vi "Variable glob Leybold.vi"() -> ()   [LabVIEW 2022 SP3]
panel:
  in  "Donnees Leybold":string[](array[string])
  in  "Nom select Leybold":string[](array[string])
  in  "Selection Leybold":bool[](array[boolean])
  in  "Noms Leybold":string[](array[string])
  in  "LEYBOLD":bool
  in  "Port RS232 Leybold":refnum<visa-resource-name>[](array[refnum])
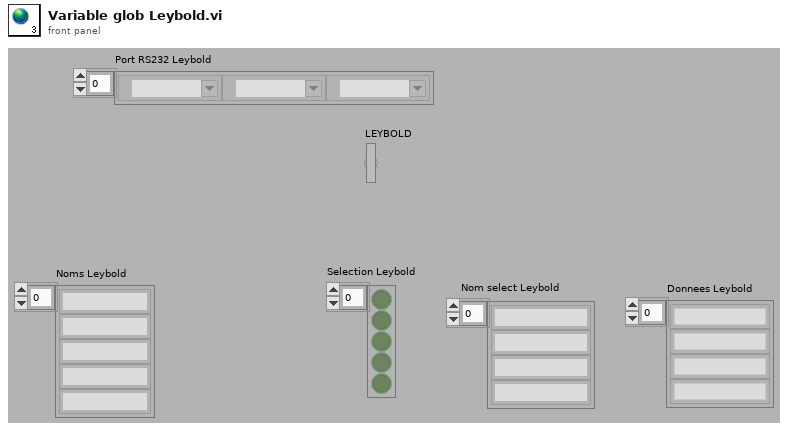
[diagram p1: front panel]
diagram:
